vi "Host_Trim.vi"(11 "string":string) -> (3 "trimmed string":string)   [LabVIEW 2018]
doc: "Use this template to build a VI to use as a subVI."
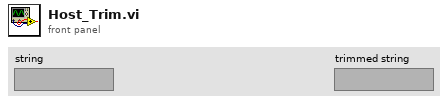
[diagram p1: front panel]
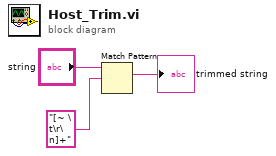
[diagram p0: block diagram]
diagram:
  n1 = Match Pattern(string="string", regular expression="[~ \t\r\n]+") -> (match substring=→"trimmed string":string)  [unwired: 1 in, 3 out]
